vi "CSE - Get number of statements.vi"(8 "error in":errorcluster, 10 "get script source (T)":bool=TRUE, 11 "CSE RefNum":T1) -> (0 "error out":errorcluster, 1 "number of statements":i32, 2 "script":string, 3 "dup CSE RefNum":T1)   [LabVIEW 2021]
doc: "This VI returns the number of statements in a parsed script. If requested (TRUE by default), it also returns the script source. Refer to the VI help for more details.\n\n::: CalcExpress Toolkit :::\nCopyright (c) 2000-2026 Konstantin Shifershteyn. All rights reserved."
uses:
  CSE Instance RefNum.ctl
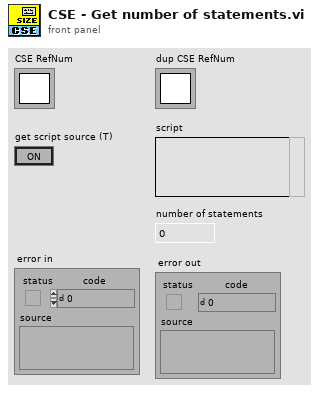
[diagram p1: front panel]
types:
  T1 = typedef "CSE Instance RefNum.ctl" = refnum<k1>
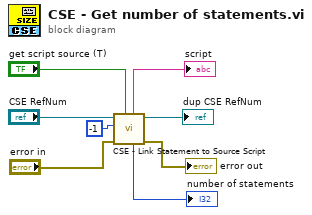
[diagram p0: block diagram]
diagram:
  n1 = call "CSE - Link Statement to Source Script.vi"("get script source (T)"="get script source (T)", "error in"="error in", "Stm Index"=-1, "CSE RefNum"="CSE RefNum") -> ("error out"=→"error out":errorcluster, "dup CSE RefNum"=→"dup CSE RefNum":T1, "size"=→"number of statements":i32, "script"=→"script":string)  [unwired: 2 in, 2 out]
